vi "Test_Run.vi"(11 "error in":errorcluster) -> ()   [LabVIEW 2026]
doc: "Test: Test_Setup, then Ticks ticks of Game_Step; at tick At[k] the key Key[k] is sent (values see Game_Step: 1 Up, 2 Down, 3 Left, 4 Right, 6 Pause, 7 Start, 8 Jump, 9 Release, 10 ReleaseV, 11 ReleaseL, 12 ReleaseR). Returns where Claude ends and the game state: X, Y (px), Mode, Room, Phase, Lives, Score, keys, torch, the highest point (Min Y), ticks in the air and all sound bits that occurred."
uses:
  Source/Engine/GH_Engine.lvlib
panel:
  out "error out":errorcluster
  out "Demo step":i32
  out "Seed out":u32
  out "Enemies out":T1(array[cluster])
  out "Sounds":i32
  out "Air ticks":i32
  out "Min Y":i32
  out "Torch out":bool
  out "KeyY":i32
  out "KeyB":i32
  out "KeyR":i32
  out "Score":i32
  out "Lives":i32
  out "Phase out":i32
  out "Room out":i32
  out "Mode":i32
  out "Y out":i32
  out "X out":i32
  in  "Keys":i32
  in  "Phase":i32=2
  in  "Torch":bool
  in  "Y":i32
  in  "X":i32
  in  "Room":i32=-1
  in  "Level":i32=1
  in  "Ticks":i32=60
  in  "Key":u16[](array[numeric])
  in  "At":i32[](array[numeric])
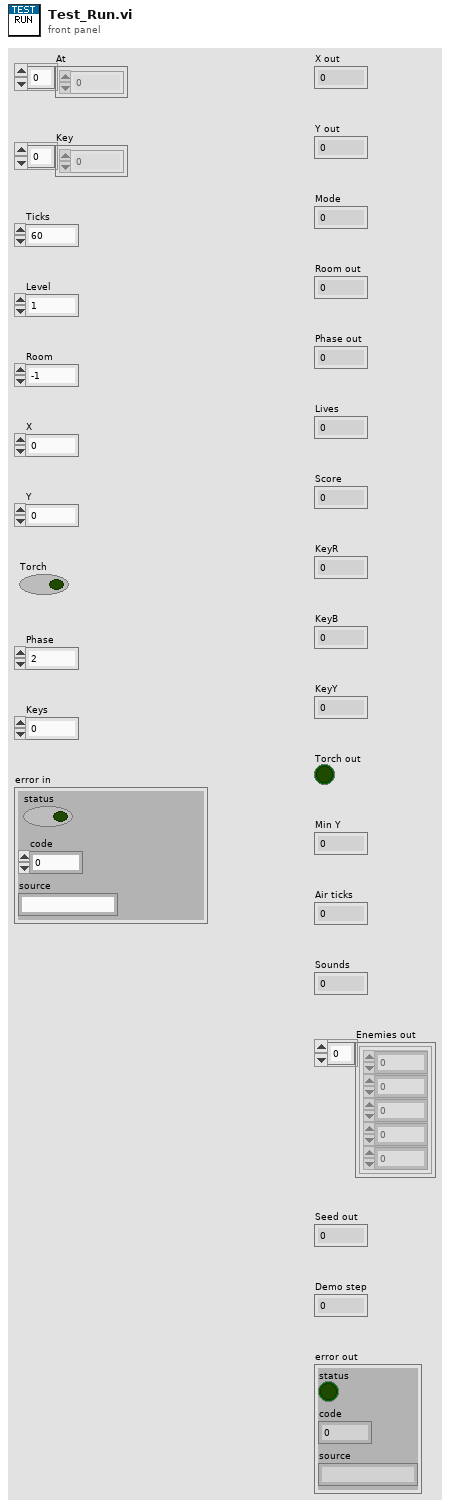
[diagram p1: front panel]
types:
  T1 = cluster{"Kind":i32, "X10":i32, "Y10":i32, "Dir":i32, "Mode":i32}[]
  T2 = cluster{"Tick":u32, "Phase":i32, "PhaseTicks":i32, "Level":i32, "Room":i32, "X10":i32, "Y10":i32, "VY10":i32, "Mode":i32, "Facing":i32, "Run":i32, "Vert":i32, "StandY":i32, "EntryX10":i32, "EntryY10":i32, "EntryMode":i32, "Lives":i32, "Score":i32, "NextLife":i32, "KeyR":i32, "KeyB":i32, "KeyY":i32, "Torch":bool, "FloorPhase":i32, "Dead":bool, "LevelStart":bool, "Quit":bool, "Sound":i32, "Seed":u32, "DemoStep":i32, "Tiles":u8[][], "World":cluster{"ID":string, "Depth":i32, "Column":i32, "Tiles":u8[][]}[], "Enemies":cluster{"Kind":i32, "X10":i32, "Y10":i32, "Dir":i32, "Mode":i32}[], "Highscores":cluster{"Score":i32, "Name":string}[], "Name":i32[], "Cursor":i32}
  T3 = cluster{"ID":string, "Depth":i32, "Column":i32, "Tiles":u8[][]}[]
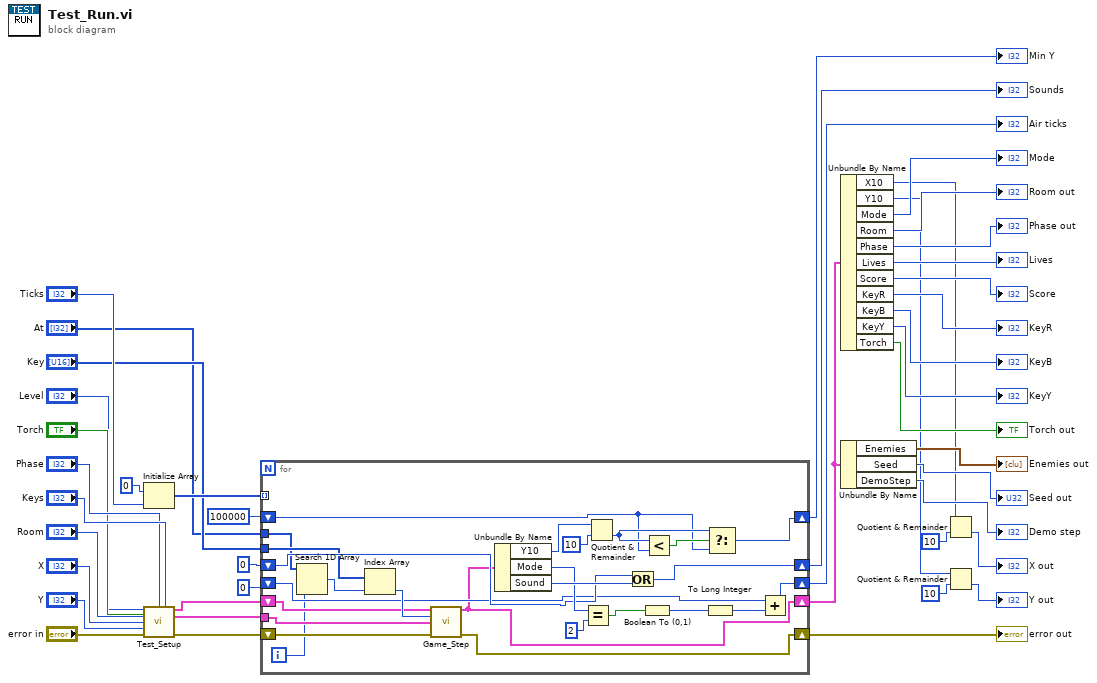
[diagram p0: block diagram]
diagram:
  n1 = Initialize Array(0, "Ticks") -> (w19:i32[])
  n2 = call "Test_Setup.vi"("Level"="Level", "Torch"="Torch", "Phase"="Phase", "Keys"="Keys", "Room"="Room", "X"="X", "Y"="Y", "error in"="error in") -> ("State"=w12:T2, "Rooms"=w13:T3, "error out"=w14:errorcluster)  [unwired: 5 in]
  n3 = for {
    tunnel: "At" -> [w44]
    tunnel: "Key" -> [w45]
    shift-right: [w52] -> w22
    shift-left: 100000 -> [w51]
    shift-right: [w54] -> w23
    shift-left: 0 -> [w53]
    shift-right: [w56] -> w24
    shift-left: 0 -> [w55]
    tunnel: w19 -> [_] mode=indexing
    tunnel: w13 -> [w46]
    shift-right: [w48] -> w20
    shift-left: w12 -> [w47]
    shift-right: [w50] -> w21
    shift-left: w14 -> [w49]
    i -> [w43]
    n4 = Search 1D Array(1D array=w44, element=w43) -> (index of element=w57:i32)  [unwired: 1 in]
    n5 = Index Array(array=w45, index=w57) -> (element=w58:u16)
    n6 = call "Game_Step.vi"("State"=w47, "Key"=w58, "Rooms"=w46, "error in"=w49) -> ("State out"=w48:T2, "error out"=w50:errorcluster)  [unwired: 10 in]
    n7 = Unbundle By Name(w48) -> ("Y10"=w59:i32, "Mode"=w60:i32, "Sound"=w61:i32)
    n8 = Equal?(x=w60, y=2) -> (x = y?=w66:bool)
    n9 = Quotient & Remainder(x=w59, y=10) -> (floor(x/y)=w63:i32)  [unwired: 1 out]
    n10 = Or(x=w55, y=w61) -> (x .or. y?=w56:i32)
    n11 = Boolean To (0,1)(Boolean=w66) -> (0, 1=w67:i16)
    n12 = Less?(x=w63, y=w51) -> (x < y?=w64:bool)
    n13 = To Long Integer(number=w67) -> (32bit integer=w68:i32)
    n14 = Select(t=w63, s=w64, f=w51) -> (s? t:f=w52:i32)
    n15 = Add(x=w53, y=w68) -> (x+y=w54:i32)
  }
  "Min Y" <- w22
  "Air ticks" <- w23
  "Sounds" <- w24
  "error out" <- w21
  n16 = Unbundle By Name(w20) -> ("X10"=w25:i32, "Y10"=w26:i32, "Mode"=→"Mode":i32, "Room"=→"Room out":i32, "Phase"=→"Phase out":i32, "Lives"=→"Lives":i32, "Score"=→"Score":i32, "KeyR"=→"KeyR":i32, "KeyB"=→"KeyB":i32, "KeyY"=→"KeyY":i32, "Torch"=→"Torch out":bool)
  n17 = Unbundle By Name(w20) -> ("Enemies"=→"Enemies out":T1, "Seed"=→"Seed out":u32, "DemoStep"=→"Demo step":i32)
  n18 = Quotient & Remainder(x=w25, y=10) -> (floor(x/y)=→"X out":i32)  [unwired: 1 out]
  n19 = Quotient & Remainder(x=w26, y=10) -> (floor(x/y)=→"Y out":i32)  [unwired: 1 out]
